vi "VIH HelpGen - Settings - Container.vi"(6 "cmd (get)":enum16{"get", "set", "load", "save"}(ring), 8 "error in":errorcluster, 10 "Settings in":T1) -> (0 "error out":errorcluster, 2 "Settings out":T1)   [LabVIEW 2014]
doc: "::: VI Helpeks :::\nCopyright (c) 2000-2026 Konstantin Shifershteyn. All rights reserved."
uses:
  <vilib>/Utility/config.llb/Read Key (Boolean).vi
  <vilib>/Utility/config.llb/Read Key (I32).vi
  <vilib>/Utility/config.llb/Read Key (String).vi
  <vilib>/Utility/config.llb/Write Key (Boolean).vi
  <vilib>/Utility/config.llb/Write Key (I32).vi
  <vilib>/Utility/config.llb/Write Key (String).vi
  <vilib>/Utility/config.llb/NI_LVConfig.lvlib
panel:
  # "VI Helpeks\nCopyright (c) 2012-2026 Konstantin Shifershteyn"
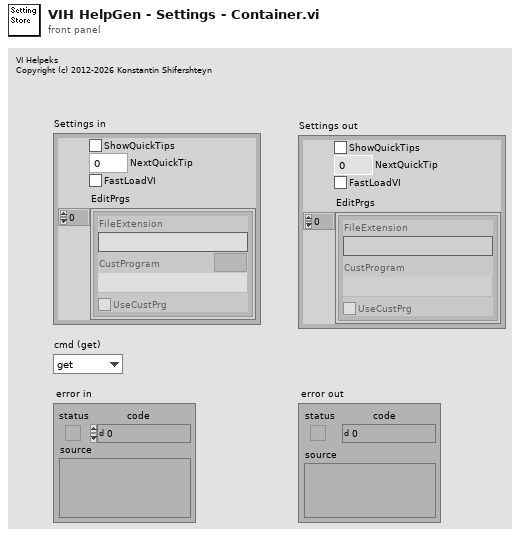
[diagram p1: front panel]
types:
  T1 = cluster{"ShowQuickTips":bool, "NextQuickTip":i32, "FastLoadVI":bool, "EditPrgs ":cluster{"FileExtension":string, "CustProgram":path, "UseCustPrg":bool}[]}
  T2 = typedef "NI_LVConfig.lvlib/Config Data RefNum.ctl" = refnum<k1>
  T3 = cluster{"FileExtension":string, "CustProgram":path, "UseCustPrg":bool}[]
  T4 = cluster{"FileExtension":string, "CustProgram":path, "UseCustPrg":bool}
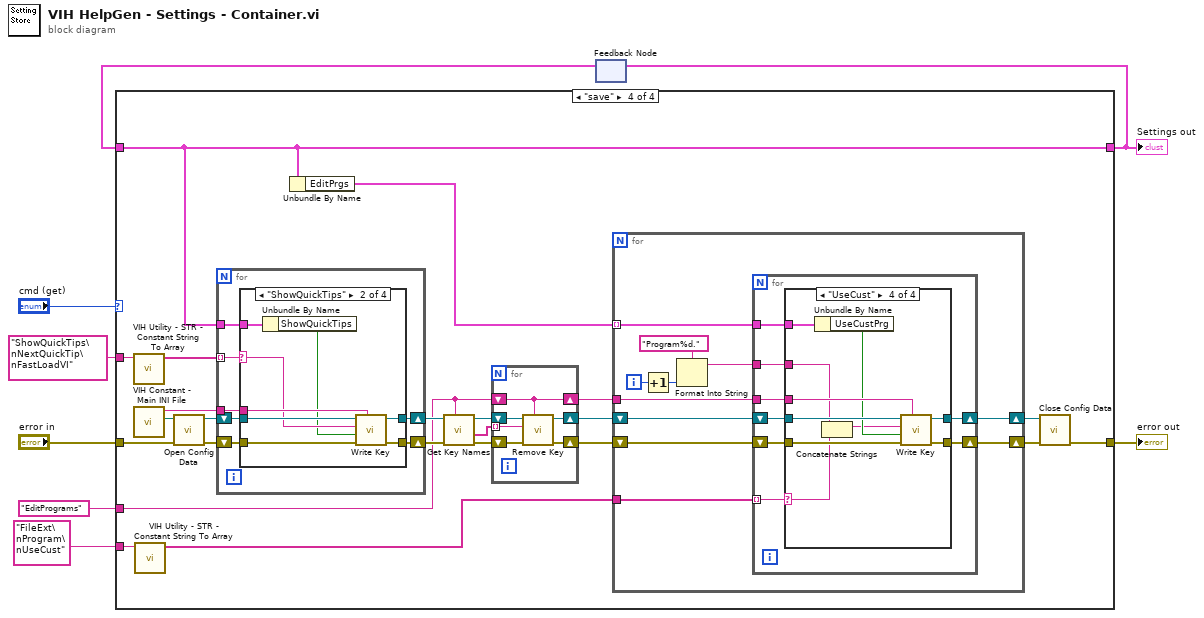
[diagram p0: block diagram]
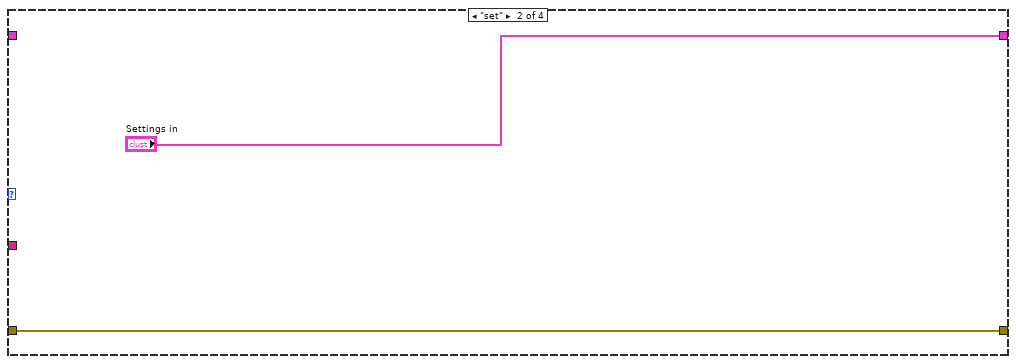
[diagram p3: hidden frame]
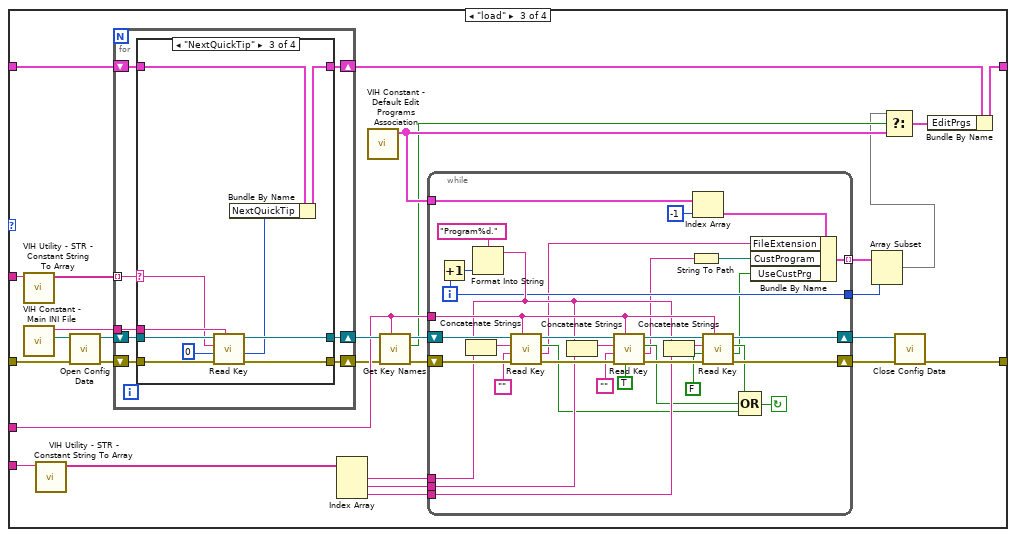
[diagram p4: hidden frame]
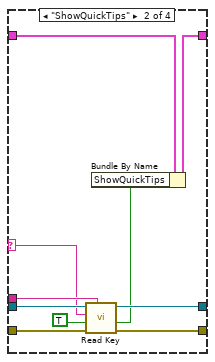
[diagram p6: hidden frame]
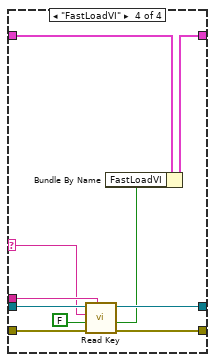
[diagram p7: hidden frame]
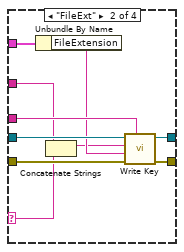
[diagram p9: hidden frame]
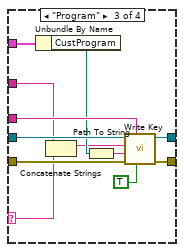
[diagram p10: hidden frame]
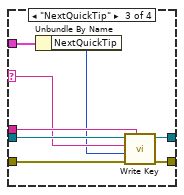
[diagram p12: hidden frame]
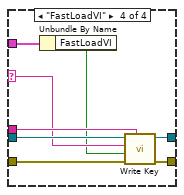
[diagram p13: hidden frame]
diagram:
  n1 = feedback #1() -> (w6:T1)  [unwired: 1 in]
  n2 = case shown="\"save\"" "cmd (get)" {
    tunnel: [w10 "Settings in" w23 w126] -> w7
    tunnel: w6 -> [w10 _ w33 w126]
    tunnel: "error in" -> [w9 w11 w36 w139]
    tunnel: [w9 w11 w35 w138] -> w4
    tunnel: "ShowQuickTips\nNextQuickTip\nFastLoadVI" -> [_ _ w34 w137]
    tunnel: "EditPrograms" -> [_ _ w19 w122]
    tunnel: "FileExt\nProgram\nUseCust" -> [_ _ w30 w128]
    frame "get" {
    }
    frame "set" {
    }
    frame "load" {
      n3 = call "VIH Utility - STR - Constant String To Array.vi"("String in"=w34) -> ("Array out"=w37:string[])  [unwired: 10 in]
      n4 = call "VIH Constant - Main INI File.vi"() -> ("Main INI File"=w41:path, "Section"=w38:string)  [unwired: 10 in]
      n5 = call "VIH Utility - STR - Constant String To Array.vi"("String in"=w30) -> ("Array out"=w29:string[])  [unwired: 10 in]
      n6 = call <vilib>:"Open Config Data.vi"("error in (no error)"=w36, "configuration file path"=w41) -> ("error out"=w39:errorcluster, "refnum"=w40:T2)  [unwired: 7 in, 1 out]
      n7 = for {
        tunnel: w38 -> [w80]
        shift-right: [w82] -> w21
        shift-left: w40 -> [w84]
        shift-right: [w81] -> w18
        shift-left: w39 -> [w83]
        tunnel: w37 -> [w79] mode=indexing
        shift-right: [w78] -> w22
        shift-left: w33 -> [w77]
        n8 = case shown="\"NextQuickTip\"" w79 {
          selector: w79 -> [_ w92 w102 w112]
          tunnel: w84 -> [w86 w97 w107 w117]
          tunnel: w83 -> [w87 w96 w106 w116]
          tunnel: [w86 w95 w105 w115] -> w82
          tunnel: [w87 w94 w104 w114] -> w81
          tunnel: w80 -> [_ w93 w103 w113]
          tunnel: [w85 w90 w100 w110] -> w78
          tunnel: w77 -> [w85 w91 w101 w111]
          frame Default {
          }
          frame "ShowQuickTips" {
            n9 = call-poly <vilib>:"Read Key.vi"("section"=w93, "error in (no error)"=w96, "default value"=TRUE, "key"=w92, "refnum"=w97) -> ("error out"=w94:errorcluster, "value"=w89:bool, "refnum out"=w95:T2)  [unwired: 3 in, 1 out]
            n10 = Bundle By Name(cluster=w91, "ShowQuickTips"=w89) -> (w90:T1)
          }
          frame "NextQuickTip" {
            n11 = call-poly <vilib>:"Read Key.vi"("section"=w103, "error in (no error)"=w106, "default value"=0, "key"=w102, "refnum"=w107) -> ("error out"=w104:errorcluster, "value"=w99:i32, "refnum out"=w105:T2)  [unwired: 3 in, 1 out]
            n12 = Bundle By Name(cluster=w101, "NextQuickTip"=w99) -> (w100:T1)
          }
          frame "FastLoadVI" {
            n13 = call-poly <vilib>:"Read Key.vi"("section"=w113, "error in (no error)"=w116, "default value"=FALSE, "key"=w112, "refnum"=w117) -> ("error out"=w114:errorcluster, "value"=w109:bool, "refnum out"=w115:T2)  [unwired: 3 in, 1 out]
            n14 = Bundle By Name(cluster=w111, "FastLoadVI"=w109) -> (w110:T1)
          }
        }
      }
      n15 = Index Array(array=w29) -> (element #1=w28:string, element #2=w27:string, element #3=w26:string)  [unwired: 3 in]
      n16 = call "VIH Constant - Default Edit Programs Association.vi"() -> ("Default Edit Programs"=w16:T3)  [unwired: 11 in]
      n17 = call <vilib>:"Get Key Names.vi"("section"=w19, "error in (no error)"=w18, "refnum"=w21) -> ("error out"=w17:errorcluster, "section exists?"=w15:bool, "refnum out"=w20:T2)  [unwired: 5 in, 1 out]
      n18 = while {
        shift-right: [w73] -> w32
        shift-left: w20 -> [w76]
        shift-right: [w69] -> w31
        shift-left: w17 -> [w72]
        tunnel: w19 -> [w68]
        tunnel: w28 -> [w62]
        tunnel: w27 -> [w61]
        tunnel: w26 -> [w58]
        tunnel: [w51] -> w25 mode=indexing
        tunnel: [w50] -> w24
        tunnel: w16 -> [w43]
        i -> [w50]
        stop <- w54 continue-if-true
        n19 = Increment(x=w50) -> (x+1=w64:i32)
        n20 = Format Into String(format string="Program%d.", w64) -> (resulting string=w56:string)  [unwired: 2 in, 1 out]
        n21 = Concatenate Strings(w56, w62) -> (w60:string)
        n22 = call-poly <vilib>:"Read Key.vi"("section"=w68, "error in (no error)"=w72, "default value"="", "key"=w60, "refnum"=w76) -> ("error out"=w71:errorcluster, "value"=w49:string, "found?"=w52:bool, "refnum out"=w75:T2)  [unwired: 3 in]
        n23 = Concatenate Strings(w56, w61) -> (w59:string)
        n24 = call-poly <vilib>:"Read Key.vi"("read raw string? (F)"=TRUE, "section"=w68, "error in (no error)"=w71, "default value"="", "key"=w59, "refnum"=w75) -> ("error out"=w70:errorcluster, "value"=w48:string, "found?"=w53:bool, "refnum out"=w74:T2)  [unwired: 2 in]
        n25 = Concatenate Strings(w56, w58) -> (w57:string)
        n26 = String To Path(string=w48) -> (path=w45:path)
        n27 = Index Array(array=w43, index=-1) -> (element=w42:T4)
        n28 = call-poly <vilib>:"Read Key.vi"("section"=w68, "error in (no error)"=w70, "default value"=FALSE, "key"=w57, "refnum"=w74) -> ("error out"=w69:errorcluster, "value"=w47:bool, "found?"=w55:bool, "refnum out"=w73:T2)  [unwired: 3 in]
        n29 = Compound Arithmetic op=OR(w55, w53, w52) -> (w54:bool)
        n30 = Bundle By Name(cluster=w42, "FileExtension"=w49, "CustProgram"=w45, "UseCustPrg"=w47) -> (w51:T4)
      }
      n31 = Array Subset(array=w25, length=w24) -> (w13:T3)  [unwired: 1 in]
      n32 = Select(t=w13, s=w15, f=w16) -> (s? t:f=w14:T3)
      n33 = call <vilib>:"Close Config Data.vi"("error in (no error)"=w31, "refnum"=w32) -> ("error out"=w35:errorcluster)  [unwired: 8 in, 1 out]
      n34 = Bundle By Name(cluster=w22, "EditPrgs"=w14) -> (w23:T1)
    }
    frame "save" {
      n35 = call "VIH Utility - STR - Constant String To Array.vi"("String in"=w137) -> ("Array out"=w133:string[])  [unwired: 10 in]
      n36 = call "VIH Constant - Main INI File.vi"() -> ("Main INI File"=w140:path, "Section"=w134:string)  [unwired: 10 in]
      n37 = call "VIH Utility - STR - Constant String To Array.vi"("String in"=w128) -> ("Array out"=w127:string[])  [unwired: 10 in]
      n38 = call <vilib>:"Open Config Data.vi"("error in (no error)"=w139, "configuration file path"=w140) -> ("error out"=w135:errorcluster, "refnum"=w136:T2)  [unwired: 7 in, 1 out]
      n39 = for {
        shift-right: [w204] -> w130
        shift-left: w136 -> [w206]
        shift-right: [w203] -> w129
        shift-left: w135 -> [w205]
        tunnel: w134 -> [w202]
        tunnel: w133 -> [w201] mode=indexing
        tunnel: w126 -> [w200]
        n40 = case shown="\"ShowQuickTips\"" w201 {
          selector: w201 -> [_ w210 w218 w226]
          tunnel: w206 -> [w208 w216 w224 w232]
          tunnel: w205 -> [w207 w215 w223 w231]
          tunnel: [w208 w214 w222 w230] -> w204
          tunnel: [w207 w213 w221 w229] -> w203
          tunnel: w202 -> [_ w212 w220 w228]
          tunnel: w200 -> [_ w211 w219 w227]
          frame Default {
          }
          frame "ShowQuickTips" {
            n41 = Unbundle By Name(w211) -> ("ShowQuickTips"=w209:bool)
            n42 = call-poly <vilib>:"Write Key.vi"("section"=w212, "error in (no error)"=w215, "value"=w209, "key"=w210, "refnum"=w216) -> ("error out"=w213:errorcluster, "refnum out"=w214:T2)  [unwired: 4 in, 1 out]
          }
          frame "NextQuickTip" {
            n43 = Unbundle By Name(w219) -> ("NextQuickTip"=w217:i32)
            n44 = call-poly <vilib>:"Write Key.vi"("section"=w220, "error in (no error)"=w223, "value"=w217, "key"=w218, "refnum"=w224) -> ("error out"=w221:errorcluster, "refnum out"=w222:T2)  [unwired: 4 in, 1 out]
          }
          frame "FastLoadVI" {
            n45 = Unbundle By Name(w227) -> ("FastLoadVI"=w225:bool)
            n46 = call-poly <vilib>:"Write Key.vi"("section"=w228, "error in (no error)"=w231, "value"=w225, "key"=w226, "refnum"=w232) -> ("error out"=w229:errorcluster, "refnum out"=w230:T2)  [unwired: 4 in, 1 out]
          }
        }
      }
      n47 = Unbundle By Name(w126) -> ("EditPrgs"=w125:T3)
      n48 = call <vilib>:"Get Key Names.vi"("section"=w122, "error in (no error)"=w129, "refnum"=w130) -> ("error out"=w123:errorcluster, "key names"=w118:string[], "refnum out"=w124:T2)  [unwired: 5 in, 1 out]
      n49 = for {
        shift-right: [w145] -> w121
        shift-left: w122 -> [w145]
        shift-right: [w142] -> w120
        shift-left: w124 -> [w146]
        shift-right: [w143] -> w119
        shift-left: w123 -> [w144]
        tunnel: w118 -> [w141] mode=indexing
        n50 = call <vilib>:"Remove Key.vi"("section"=w145, "error in (no error)"=w144, "key"=w141, "refnum"=w146) -> ("error out"=w143:errorcluster, "refnum out"=w142:T2)  [unwired: 5 in, 1 out]
      }
      n51 = for {
        shift-right: [w155] -> w132
        shift-left: w120 -> [w157]
        shift-right: [w154] -> w131
        shift-left: w119 -> [w156]
        tunnel: w127 -> [w153]
        tunnel: w125 -> [w152] mode=indexing
        tunnel: w121 -> [w151]
        i -> [w150]
        n52 = Increment(x=w150) -> (x+1=w149:i32)
        n53 = Format Into String(format string="Program%d.", w149) -> (resulting string=w147:string)  [unwired: 2 in, 1 out]
        n54 = for {
          shift-right: [w163] -> w155
          shift-left: w157 -> [w165]
          shift-right: [w162] -> w154
          shift-left: w156 -> [w164]
          tunnel: w153 -> [w161] mode=indexing
          tunnel: w152 -> [w160]
          tunnel: w151 -> [w159]
          tunnel: w147 -> [w158]
          n55 = case shown="\"UseCust\"" w161 {
            selector: w161 -> [_ w168 w180 w190]
            tunnel: w165 -> [w167 w177 w189 w199]
            tunnel: w164 -> [w166 w176 w188 w198]
            tunnel: [w167 w175 w187 w197] -> w163
            tunnel: [w166 w174 w186 w196] -> w162
            tunnel: w159 -> [_ w173 w185 w195]
            tunnel: w160 -> [_ w172 w184 w194]
            tunnel: w158 -> [_ w169 w181 w191]
            frame Default {
            }
            frame "FileExt" {
              n56 = Unbundle By Name(w172) -> ("FileExtension"=w171:string)
              n57 = Concatenate Strings(w169, w168) -> (w170:string)
              n58 = call-poly <vilib>:"Write Key.vi"("section"=w173, "error in (no error)"=w176, "value"=w171, "key"=w170, "refnum"=w177) -> ("error out"=w174:errorcluster, "refnum out"=w175:T2)  [unwired: 4 in, 1 out]
            }
            frame "Program" {
              n59 = Unbundle By Name(w184) -> ("CustProgram"=w183:path)
              n60 = Concatenate Strings(w181, w180) -> (w182:string)
              n61 = Path To String(path=w183) -> (string=w179:string)
              n62 = call-poly <vilib>:"Write Key.vi"("write raw string? (F)"=TRUE, "section"=w185, "error in (no error)"=w188, "value"=w179, "key"=w182, "refnum"=w189) -> ("error out"=w186:errorcluster, "refnum out"=w187:T2)  [unwired: 3 in, 1 out]
            }
            frame "UseCust" {
              n63 = Unbundle By Name(w194) -> ("UseCustPrg"=w193:bool)
              n64 = Concatenate Strings(w191, w190) -> (w192:string)
              n65 = call-poly <vilib>:"Write Key.vi"("section"=w195, "error in (no error)"=w198, "value"=w193, "key"=w192, "refnum"=w199) -> ("error out"=w196:errorcluster, "refnum out"=w197:T2)  [unwired: 4 in, 1 out]
            }
          }
        }
      }
      n66 = call <vilib>:"Close Config Data.vi"("error in (no error)"=w131, "refnum"=w132) -> ("error out"=w138:errorcluster)  [unwired: 8 in, 1 out]
    }
  }
  "Settings out" <- w7
  "error out" <- w4
  n67 = feedback-in #1(w7) -> ()
